vi "D4xxx Set Sense and Guard.vi"(8 "error in":errorcluster, 9 "Guard (0: Local)":u16(ring) items=["Local", "Remote"], 10 "Sense (0: Local)":u16(ring) items=["Local", "Remote"], 11 "4808":refnum<visa-resource-name>) -> (0 "error out":errorcluster, 3 "Session Out":refnum<visa-resource-name>)   [LabVIEW 2009]
doc: "Set Guard and Sense of Datron 4xxx series calibrators. False means local, True means remote."
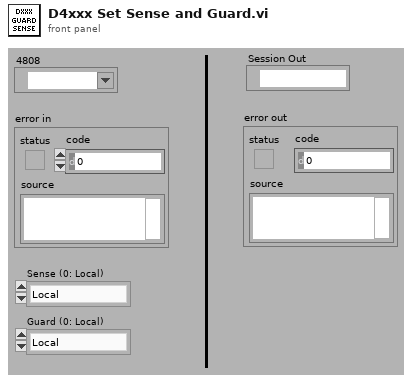
[diagram p1: front panel]
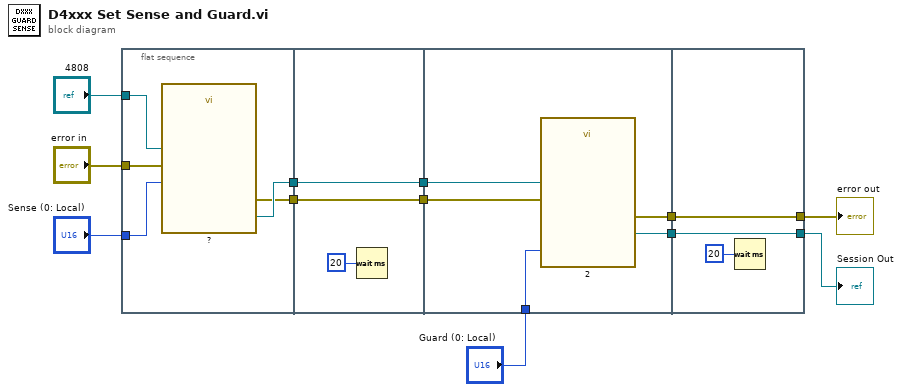
[diagram p0: block diagram]
diagram:
  n1 = flat-sequence {
    tunnel: "4808" -> [w17]
    tunnel: [w16] -> w6
    tunnel: "error in" -> [w15]
    tunnel: [w14] -> w5
    tunnel: "Sense (0: Local)" -> [w13]
    tunnel: [w20] -> w4
    tunnel: w6 -> [w20]
    tunnel: [w18] -> w3
    tunnel: w5 -> [w18]
    tunnel: w4 -> [w25]
    tunnel: w3 -> [w24]
    tunnel: "Guard (0: Local)" -> [w21]
    tunnel: [w23] -> w2
    tunnel: [w22] -> w1
    tunnel: [w27] -> w12
    tunnel: [w28] -> w11
    tunnel: w2 -> [w28]
    tunnel: w1 -> [w27]
    frame #0 {
      n2 = call "?"("Session In"=w17, "sense"=w13, "error in"=w15) -> ("Session Out"=w16:refnum<visa-resource-name>, "error out"=w14:errorcluster)  [unwired: 23 in]
    }
    frame #1 {
      n3 = Wait (ms)(milliseconds to wait=u32 20 ("millisecond multiple")) -> ()  [unwired: 1 out]
    }
    frame #2 {
      n4 = call "2"("Session In"=w25, "guard"=w21, "error in"=w24) -> ("Session Out"=w22:refnum<visa-resource-name>, "error out"=w23:errorcluster)  [unwired: 23 in]
    }
    frame #3 {
      n5 = Wait (ms)(milliseconds to wait=u32 20 ("millisecond multiple")) -> ()  [unwired: 1 out]
    }
  }
  "Session Out" <- w12
  "error out" <- w11
